vi "Transmitter_Example_V3.vi"() -> ()   [LabVIEW 2022 SP3]
uses:
  <instrlib>/niUSRP/niUSRP Write Tx Data (CDB Cluster).vi
panel:
  in  "Modulation parameter LP":T1
  in  "String Critical Data 2":string="Critical Dataaaaa\nCritical Dataaaaa\nCritical Dataaaaa\nCritical Dataaaaa\nCritical Dataaaaa\nNon Critical Data\nNon Critical Data\nNon Critical Data\nNon Critical Data\nNon Critical Data"
  in  "milliseconds to wait":u32=100
  in  "OFDM 4QAM / 16QAM":bool
  out "AuxString 2":string
  out "AuxString":string
  in  "Previous Button":bool caption="Both Critical and Non Critical\nData must be equal size."
  in  "New Critical Data":string="Non Critical Data\nNon Critical Data\nNon Critical Data\nNon Critical Data\nNon Critical Data"
  in  "New Non Critical Data":string="Critical Dataaaaa\nCritical Dataaaaa\nCritical Dataaaaa\nCritical Dataaaaa\nCritical Dataaaaa"
  out "Frame Duration 2":dbl format="%#_6p"
  in  "Alpha":dbl=0.05 min=0.0 max=1.0 step=0.05
  out "Bits length 2":i32
  in  "String Critical Data":string="Non Critical Data\nNon Critical Data\nNon Critical Data\nNon Critical Data\nNon Critical Data\n"
  in  "Modulation parameter HP":T1
  out "Bits length":i32
  out "Frame Duration":dbl format="%#_6p"
  out "Waveform Graph":cluster{"t0":dbl, "dt":dbl, "Y":dbl[]}(graph)
  in  "stop":bool
  in  "String Non Critical Data":string="Critical Dataaaaa\nCritical Dataaaaa\nCritical Dataaaaa\nCritical Dataaaaa\nCritical Dataaaaa\n"
  out "USRP CoercedParamters":T2={"coerced IQ rate"=100000.0, "coerced carrier frequency"=100000.0, "coerced gain"=0.0} {"coerced gain" format="%#_6f"; "coerced carrier frequency" format="%#_6p"; "coerced IQ rate" format="%#_6p"}
  out "error out":errorcluster
  in  "error in (no error)":errorcluster
  in  "USRP ControledParameters":T3={"active antenna"="TX1", "gain"=10.0, "carrier frequency"=2400000000.0, "IQ rate"=2000000.0} {"IQ rate" format="%#_6p"; "carrier frequency" format="%#_6p"; "gain" format="%#_6f"}
  in  "device names":refnum<k15>="RIO0"
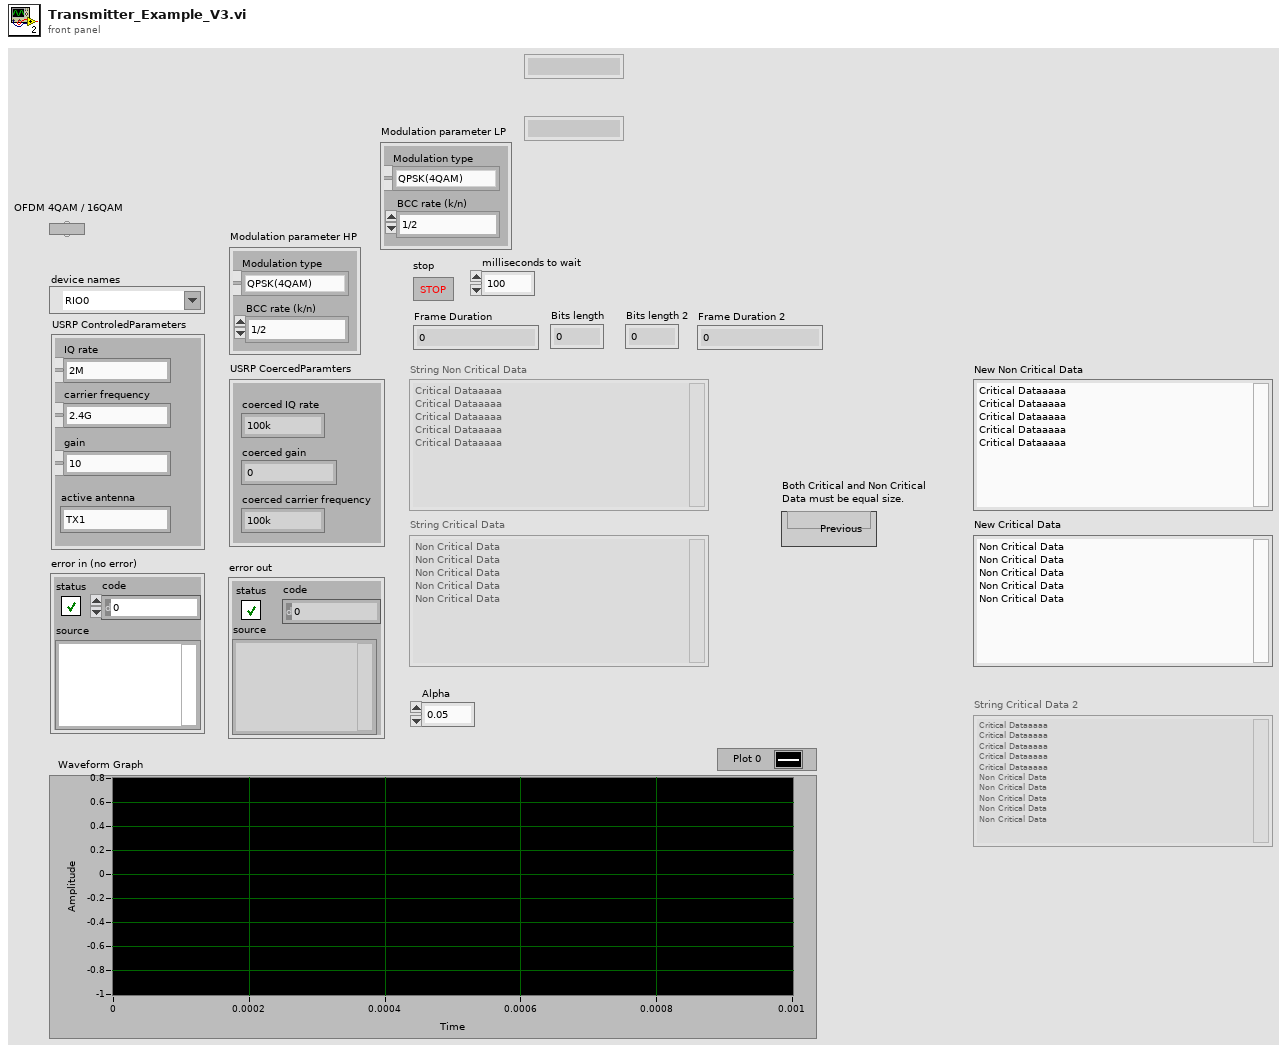
[diagram p1: front panel]
types:
  T1 = cluster{"Modulation type":enum16{"QPSK(4QAM)", "64QAM", "16QAM", "BPSK"}, "BCC rate (k/n)":enum16{"1/2", "2/3", "3/4"}}
  T2 = cluster{"coerced IQ rate":dbl, "coerced carrier frequency":dbl, "coerced gain":dbl}
  T3 = cluster{"active antenna":string, "gain":dbl, "carrier frequency":dbl, "IQ rate":dbl}
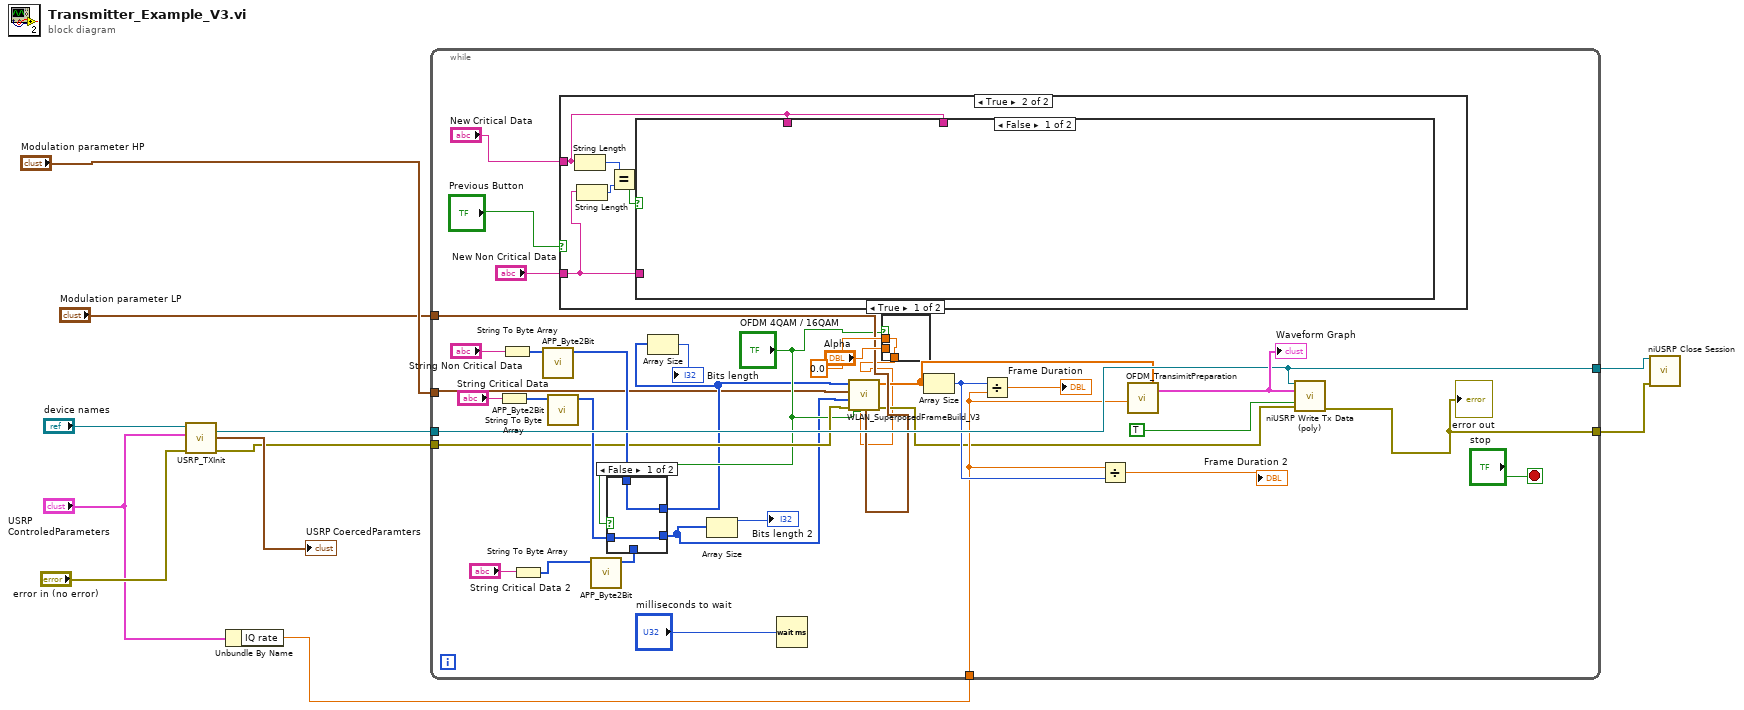
[diagram p0: block diagram]
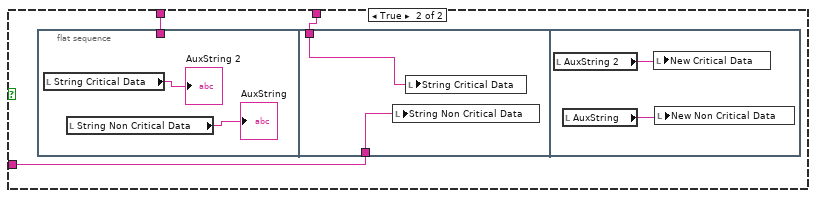
[diagram p5: hidden frame]
diagram:
  n1 = call "USRP_TXInit.vi"("device names"="device names", "USRP ControledParameters"="USRP ControledParameters", "error in (no error)"="error in (no error)") -> ("session handle out"=w9:refnum<k15>, "USRP CoercedParamters"=→"USRP CoercedParamters":T2, "error out"=w6:errorcluster)  [unwired: 5 in]
  n2 = Unbundle By Name("USRP ControledParameters") -> ("IQ rate"=w3:dbl)
  n3 = while {
    tunnel: w9 -> [w41]
    tunnel: "Modulation parameter HP" -> [w13]
    tunnel: w6 -> [w20]
    tunnel: w3 -> [w35]
    tunnel: [w41] -> w5
    tunnel: [w40] -> w4
    tunnel: "Modulation parameter LP" -> [w19]
    stop <- "stop" stop-if-true
    n4 = String To Byte Array(string="String Critical Data") -> (unsigned byte array=w37:u8[])
    n5 = String To Byte Array(string="String Non Critical Data") -> (unsigned byte array=w38:u8[])
    n6 = String To Byte Array(string="String Critical Data 2") -> (unsigned byte array=w25:u8[])
    n7 = call "APP_Byte2Bit.vi"("input byte stream"=w38) -> ("output bit stream"=w22:i8[])  [unwired: 10 in]
    n8 = call "APP_Byte2Bit.vi"("input byte stream"=w37) -> ("output bit stream"=w24:i8[])  [unwired: 10 in]
    n9 = case shown="True" "Previous Button" {
      tunnel: "New Non Critical Data" -> [_ w56]
      tunnel: "New Critical Data" -> [_ w52]
      frame False {
      }
      frame True {
        n10 = String Length(string=w52) -> (length=w55:i32)
        n11 = String Length(string=w56) -> (length=w54:i32)
        n12 = Equal?(x=w55, y=w54) -> (x = y?=w53:bool)
        n13 = case shown="False" w53 {
          tunnel: w56 -> [_ w59]
          tunnel: w52 -> [_ w58]
          tunnel: w52 -> [_ w57]
          frame False {
          }
          frame True {
            n14 = flat-sequence {
              tunnel: w57 -> [_]
              tunnel: w59 -> [w63]
              tunnel: w58 -> [w62]
              frame #0 {
                n15 = local read "String Critical Data"() -> (→"AuxString 2":string)
                n16 = local read "String Non Critical Data"() -> (→"AuxString":string)
              }
              frame #1 {
                n17 = local write "String Non Critical Data"(w63) -> ()
                n18 = local write "String Critical Data"(w62) -> ()
              }
              frame #2 {
                n19 = local read "AuxString 2"() -> (w64:string)
                n20 = local read "AuxString"() -> (w65:string)
                n21 = local write "New Critical Data"(w64) -> ()
                n22 = local write "New Non Critical Data"(w65) -> ()
              }
            }
          }
        }
      }
    }
    n23 = call "APP_Byte2Bit.vi"("input byte stream"=w25) -> ("output bit stream"=w23:i8[])  [unwired: 10 in]
    n24 = case shown="False" "OFDM 4QAM / 16QAM" {
      tunnel: [w48 w49] -> w12
      tunnel: w24 -> [w48 _]
      tunnel: w23 -> [_ w49]
      tunnel: [w47 w49] -> w14
      tunnel: w22 -> [w47 _]
      frame False {
      }
      frame True {
      }
    }
    n25 = Array Size(array=w14) -> (size(s)=→"Bits length":i32)
    n26 = Array Size(array=w12) -> (size(s)=→"Bits length 2":i32)
    n27 = Wait (ms)(milliseconds to wait="milliseconds to wait") -> ()  [unwired: 1 out]
    n28 = case shown="True" "OFDM 4QAM / 16QAM" {
      tunnel: [w50 w51] -> w15
      tunnel: "Alpha" -> [_ w51]
      tunnel: 0.0 ("Alpha 2") -> [w50 _]
      frame True {
      }
      frame False {
      }
    }
    n29 = call "WLAN_SuperposedFrameBuild_V3.vi"("Modulation parameter LP"=w19, "OFDMON"="OFDM 4QAM / 16QAM", "Alpha"=w15, "error in (no error)"=w20, "data in 2"=w12, "Modulation parameter HP"=w13, "data in"=w14) -> ("error out"=w17:errorcluster, "output array"=w16:cdb[])  [unwired: 3 in]
    n30 = Array Size(array=w16) -> (size(s)=w36:i32)
    n31 = Divide(x=w36, y=w35) -> (x/y=→"Frame Duration":dbl)
    n32 = Divide(x=w35, y=w36) -> (x/y=→"Frame Duration 2":dbl)
    n33 = call "OFDM_TransimitPreparation.vi"("IQ rate"=w35, "array"=w16) -> ("output cluster"=w43:cluster{"t0":dbl, "dt":dbl, "Y":cdb[]})  [unwired: 9 in]
    "Waveform Graph" <- w43
    n34 = call-poly <instrlib>:"niUSRP Write Tx Data (poly).vi"("session handle"=w41, "data"=w43, "end of data?"=TRUE, "error in (no error)"=w17) -> ("error out"=w40:errorcluster)  [unwired: 10 in, 1 out]
    "error out" <- w40
  }
  n35 = call <instrlib>:"niUSRP Close Session.vi"("session handle"=w5, "error in (no error)"=w4) -> ()  [unwired: 13 in, 1 out]
